vi "Test Deserialize Null.vi"(8 "error in (no error)":errorcluster) -> (0 "error out":errorcluster)   [LabVIEW 2013]
uses:
  src/Library/Null Value.vi
  <vilib>/addons/_JKI Toolkits/Caraya/classes/Test/Test.lvclass
  src/JKI JSON Serialization.lvlib
  <vilib>/addons/_JKI Toolkits/Caraya/classes/Assert/Assert.lvclass
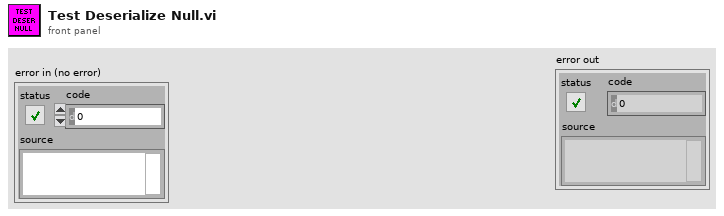
[diagram p1: front panel]
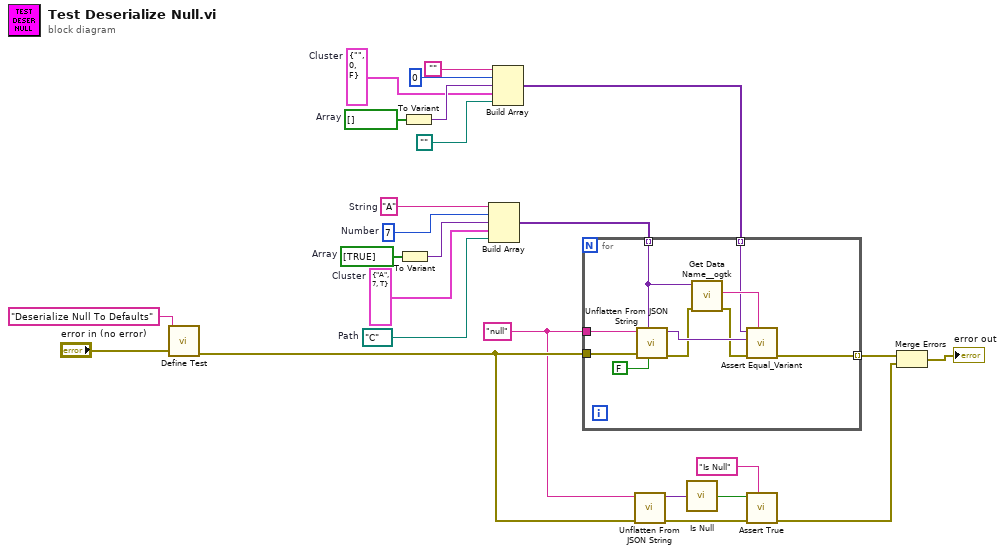
[diagram p0: block diagram]
diagram:
  w8 = cluster{"String":string, "Number":i32, bool} {"String"="", "Number"=0, FALSE}  # Cluster
  w13 = path "C:/"  # Path
  w15 = bool[] []  # Array
  w18 = cluster{"String":string, "Number":i32, bool} {"String"="A", "Number"=7, TRUE}  # Cluster
  w19 = bool[] [TRUE]  # Array
  w20 = 7  # Number
  w16 = "A"  # String
  w5 = "null" ("JSON String")
  n1 = call <vilib>:"Define Test.vi"("error in (no error)"="error in (no error)", "Label (VI Title)"="Deserialize Null To Defaults") -> ("error out"=w6:errorcluster)  [unwired: 9 in]
  n2 = To Variant(anything=w19) -> (Variant=w17:variant)
  n3 = To Variant(anything=w15) -> (Variant=w14:variant)
  n4 = Build Array(w16, w20, w17, w18, w13) -> (w21:variant[])
  n5 = Build Array("", 0 ("Number"), w14, w8, path "") -> (w11:variant[])
  n6 = for {
    tunnel: w5 -> [w35]
    tunnel: [w29] -> w22 mode=indexing
    tunnel: w6 -> [w28]
    tunnel: w21 -> [w27] mode=indexing
    tunnel: w11 -> [w26] mode=indexing
    n7 = call "Unflatten From JSON String.vi"("Nulls as Defaults (F)"=FALSE ("Nulls as Defaults (T)"), "Type and Defaults"=w27, "error in (no error)"=w28, "JSON String"=w35) -> ("error out"=w31:errorcluster, "Variant"=w33:variant)  [unwired: 6 in]
    n8 = call <userlib>:"Get Data Name__ogtk.vi"("error in (no error)"=w31, "Data"=w27) -> ("error out"=w30:errorcluster, "Data Name"=w32:string)  [unwired: 7 in, 1 out]
    n9 = call <vilib>:"Assert Equal_Variant.vi"("Label"=w32, "error in (no error)"=w30, "Y"=w33, "X"=w26) -> ("error out"=w29:errorcluster)  [unwired: 7 in]
  }
  n10 = call "Unflatten From JSON String.vi"("error in (no error)"=w6, "JSON String"=w5) -> ("error out"=w7:errorcluster, "Variant"=w4:variant)  [unwired: 8 in]
  n11 = call "Is Null.vi"("Deserialized JSON Data"=w4) -> ("Null?"=w3:bool)
  n12 = call <vilib>:"Assert True.vi"("Label"="Is Null", "error in (no error)"=w7, "True?"=w3) -> ("error out"=w2:errorcluster)  [unwired: 8 in]
  n13 = Merge Errors(w22, w2) -> (→"error out":errorcluster)
